vi "VI_List.vi"(11 "index":i32) -> (3 "Plugin VIs":refnum<vi>[](array[refnum]))   [LabVIEW 2021]
panel:
  out "error out 2":errorcluster
  out "VI Refnum":refnum<vi>
  out "error out 3":errorcluster
  out "element 2":refnum<vi>
  out "element":refnum<vi>
  out "Array":path[](array[path])
  in  "error in":errorcluster
  out "error out":errorcluster
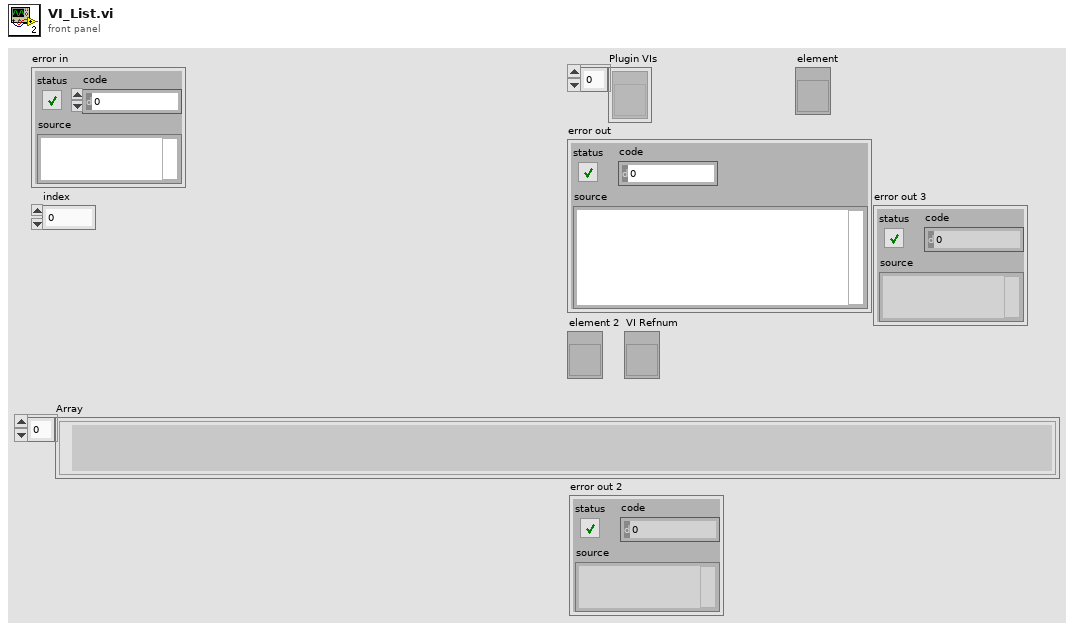
[diagram p1: front panel]
types:
  T1 = enum32{"Invalid", "Standard", "Closed", "Hidden", "Minimized", "Maximized"}
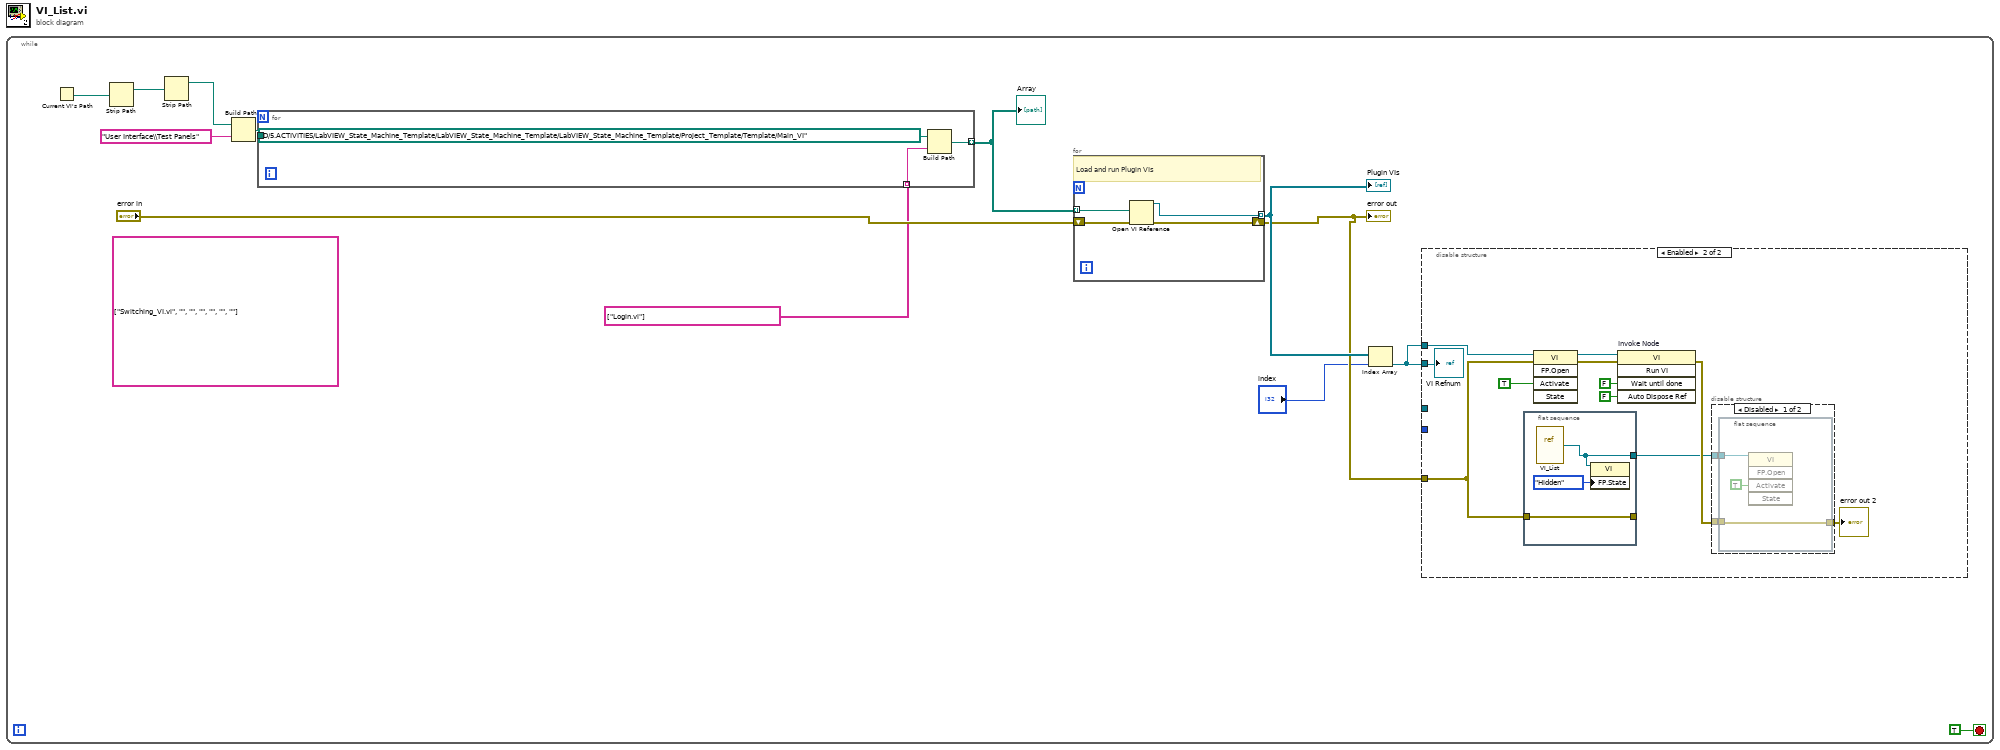
[diagram p0: block diagram]
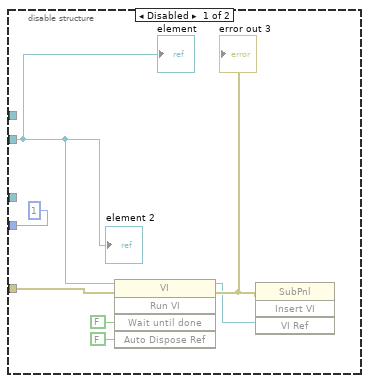
[diagram p2: hidden frame]
diagram:
  n1 = while {
    stop <- TRUE stop-if-true
    (unwired) string[] ["Switching_VI.vi", "", "", "", "", "", ""] ("name or relative path")
    n2 = Current VI's Path() -> (path=w8:path)
    n3 = Strip Path(path=w8) -> (stripped path=w9:path)  [unwired: 1 out]
    n4 = Strip Path(path=w9) -> (stripped path=w7:path)  [unwired: 1 out]
    n5 = Build Path(base path=w7, name or relative path="User Interface\\Test Panels") -> (appended path=w11:path)
    n6 = for {
      tunnel: w11 -> [_]
      tunnel: [w47] -> w10 mode=indexing
      tunnel: string[] ["Login.vi"] -> [w46] mode=indexing
      n7 = Build Path(base path=path "D:/5.ACTIVITIES/LabVIEW_State_Machine_Template/LabVIEW_State_Machine_Template/LabVIEW_State_Machine_Template/Project_Template/Template/Main_VI", name or relative path=w46) -> (appended path=w47:path)
    }
    "Array" <- w10
    n8 = for {
      tunnel: w10 -> [w49] mode=indexing
      tunnel: [w50] -> w5 mode=indexing
      shift-right: [w51] -> w4
      shift-left: "error in" -> [w48]
      # "Load and run Plugin VIs"
      n9 = Open VI Reference(vi path=w49, error in (no error)=w48) -> (vi reference=w50:refnum<vi>, error out=w51:errorcluster)  [unwired: 4 in]
    }
    "Plugin VIs" <- w5
    "error out" <- w4
    n10 = Index Array(array=w5, index="index") -> (element=w2:refnum<vi>)
    n11 = disable-structure shown="Enabled" {
      disable-tunnel: _ -> [w18 _]
      disable-tunnel: w4 -> [w17 w28]
      disable-tunnel: [1 ("index") _] -> _
      disable-tunnel: w2 -> [w14 w35]
      disable-tunnel: w2 -> [_ w34]
      frame Disabled {
        n12 = invoke class="VI" method="Run VI"(reference=w14, error in=w17, "Wait until done"=FALSE ("Wait Until Done"), "Auto Dispose Ref"=FALSE ("Auto Dispose Reference")) -> (reference out=w21:refnum<vi>, error out=w22:errorcluster)  [unwired: 1 in, 3 out]
        "error out 3" <- w22
        n13 = invoke on="Invoke Node" class="SubPnl" method="Insert VI"(error in=w22, "VI Ref"=w21) -> (reference=w16:refnum<vi>, reference out=w23:refnum<vi>, error out=w24:errorcluster)  [unwired: 1 in, 2 out]
        "element" <- w14
        "element 2" <- w14
      }
      frame Enabled {
        n14 = flat-sequence {
          tunnel: w28 -> [w43]
          tunnel: [w43] -> _
          tunnel: [w42] -> w25
          frame #0 {
            n15 = vi-ref "VI_List.vi"() -> (w42:refnum<vi>)
            n16 = property class="VI"(reference=w42, "FP.State"=T1."Hidden" ("Front Panel Window:State")) -> ()  [unwired: 1 in, 2 out]
          }
        }
        n17 = invoke class="VI" method="FP.Open"(reference=w34, error in=w28, "Activate"=TRUE ("Wait Until Done")) -> (reference out=w32:refnum<vi>, error out=w31:errorcluster)  [unwired: 2 in, 3 out]
        n18 = invoke on="Invoke Node" class="VI" method="Run VI"(reference=w32, error in=w31, "Wait until done"=FALSE ("Wait Until Done"), "Auto Dispose Ref"=FALSE ("Auto Dispose Reference")) -> (error out=w27:errorcluster)  [unwired: 1 in, 4 out]
        n19 = disable-structure shown="Disabled" {
          disable-tunnel: w27 -> [w38 _]
          disable-tunnel: [w37 _] -> w26
          disable-tunnel: w25 -> [w36 _]
          frame Disabled {
            n20 = flat-sequence {
              tunnel: [w41] -> w37
              tunnel: w38 -> [w41]
              tunnel: w36 -> [w40]
              frame #0 {
                n21 = invoke class="VI" method="FP.Open"(reference=w40, "Activate"=TRUE ("Activate?")) -> ()  [unwired: 3 in, 5 out]
              }
            }
          }
          frame Enabled {
          }
        }
        "error out 2" <- w26
        "VI Refnum" <- w35
      }
    }
  }
